vi "Main Page.vi"(8 "error in (no error)":errorcluster, 11 "Node Ptr":T1 format="%.0x") -> (0 "error out":errorcluster)   [LabVIEW 2015, in "Protection and Counter Addon System Explorer.lvlib"]
uses:
  Protection and Counter Addon System Explorer.lvlib
  <vilib>/NI Veristand/Custom Device API/Custom Device Item Ref.ctl
  <vilib>/NI/Hardware Resource Discovery/Types/Filter Type.ctl
  Shared/Types/986x.ctl
  Shared/SubVIs/GUID Lookup.vi
  <vilib>/NI Veristand/Custom Device API/NI VeriStand - Get Item Property.vi
  <vilib>/NI Veristand/Custom Device API/Get Item Property (Boolean).vi
  <vilib>/NI Veristand/Custom Device API/Get Item Property (String).vi
  <vilib>/NI Veristand/Custom Device API/Get Item Property (Dependent File).vi
  <vilib>/NI VeriStand/Custom Device API/Custom Device API.lvlib
  <vilib>/NI/Hardware Resource Discovery/NIVS Hardware Discovery.lvlib
  Shared/Protection and Counter Addon Shared.lvlib
panel:
  in  "FPGA Settings":cluster{"Section Name":string}={"Section Name"="FPGA Settings"}
  in  "RIO Browse":bool
  in  "RIO Device":string
  in  "Enable Bitfile":bool
  in  "Bitfile Path":path
  in  "Use Legacy":bool
  in  "Loop Priority":i32=100 format="%.0p"
  in  "FD Baud rate [Bd]":u64 format="%.0p"
  in  "CAN I/O Mode":u32(ring) items=["CAN 2.0", "CAN FD", "CAN FD+BRS"]
  in  "Database Settings":cluster{"Section Name":string}={"Section Name"="Database Settings"}
  in  "CAN Browse":bool
  in  "Termination":enum16{"Off", "On"}(ring)
  in  "CAN Port":string
  in  "Baud rate [Bd]":u64 format="%.0p"
  out "XNET Cluster":refnum<k21>
  out "XNET Database":refnum<k21>
  in  "SHDocVw.IWebBrowser2":refnum<k7>(container)
  in  "Header":cluster{"Section Name":string}={"Section Name"="CAN Settings"}
  in  "Name":string
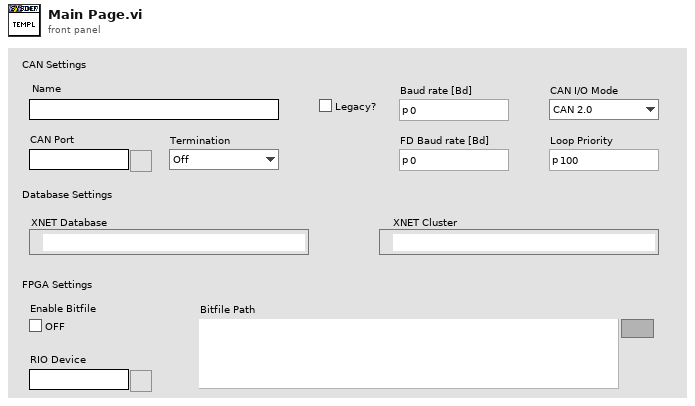
[diagram p1: front panel]
types:
  T1 = typedef "Custom Device API.lvlib/Custom Device Item Ref.ctl" = u64
  T2 = typedef "Protection and Counter Addon Shared.lvlib/986x.ctl" = cluster{"Enable":bool, "RIO Device":string, "Bitfile":path}
  T3 = typedef "Protection and Counter Addon Shared.lvlib/XNET Settings.ctl" = cluster{"Database":refnum<k21>, "Cluster":refnum<k21>, "Port":string, "Baud rate [Bd]":u64, "Termination":u32, "CAN I/O Mode":u32, "FD Baud rate [Bd]":u64, "Priority":i32, "Use Legacy":bool}
  T4 = typedef "Custom Device API.lvlib/Custom Device Item Info.ctl" = cluster{"Name":string, "Is Channel":bool, "GUID":string, "Is Waveform":bool}
  T5 = typedef "NIVS Hardware Discovery.lvlib/Filter Type.ctl" = enum16{"Device Category", "Product Name", "Ethernet", "XNET", "VISA", "FPGA", "EtherCAT Master", "DAQmx", "GPIB", "Serial"}
  T6 = typedef "Custom Device API.lvlib/Custom Device Commands.ctl" = enum16{"Default", "Item renamed", "Shutdown", "Dynamic button pressed"}
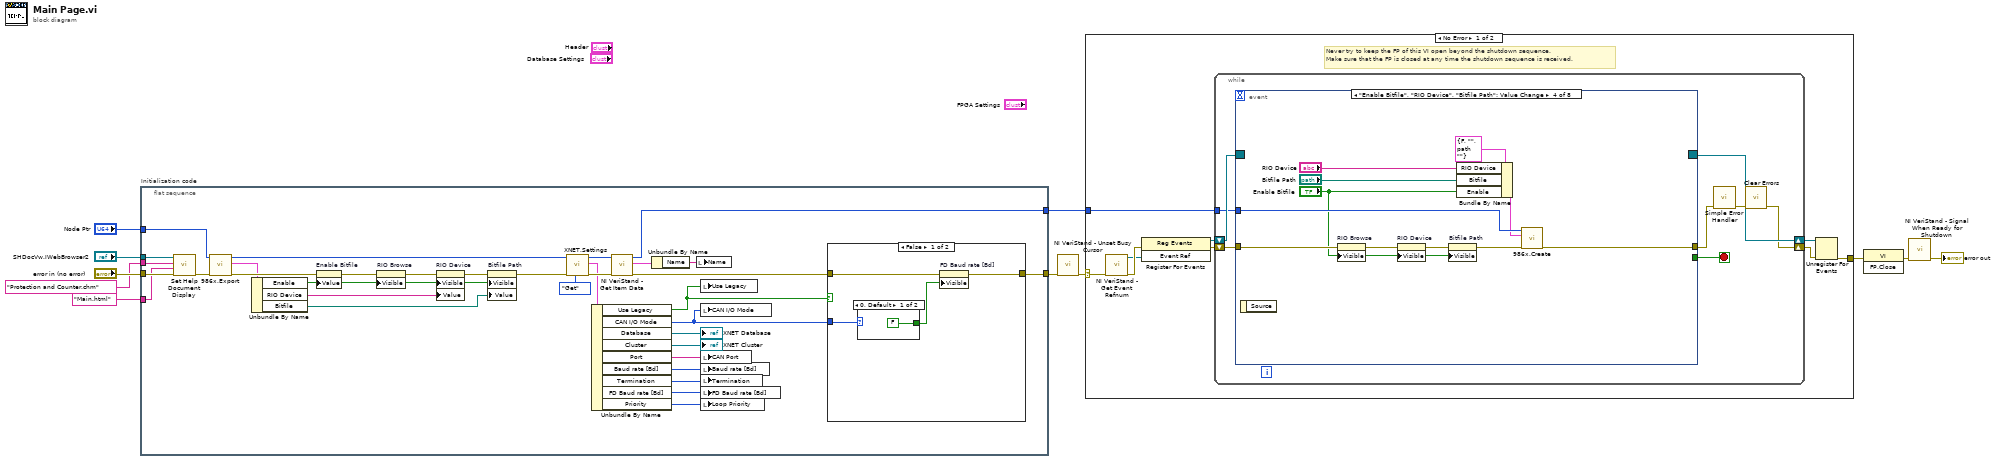
[diagram p0: block diagram]
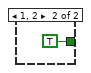
[diagram p2: hidden frame]
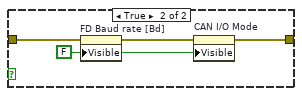
[diagram p3: hidden frame]
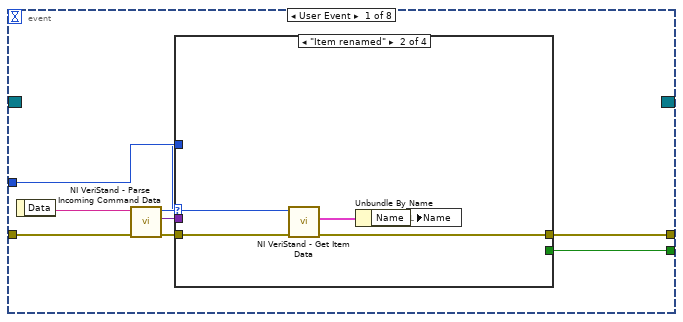
[diagram p4: hidden frame]
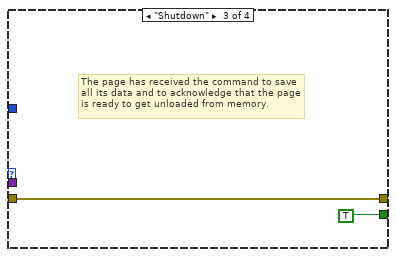
[diagram p6: hidden frame]
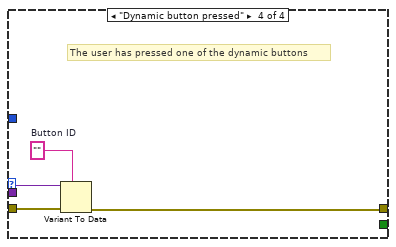
[diagram p7: hidden frame]
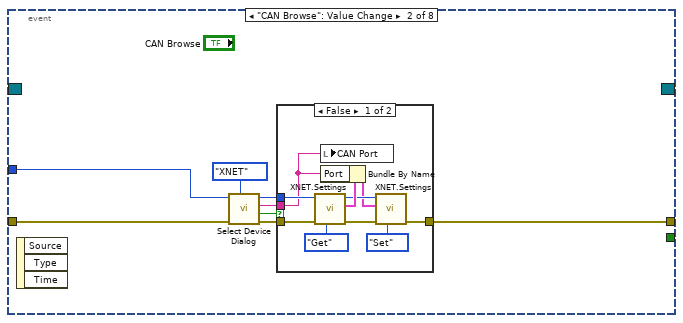
[diagram p8: hidden frame]
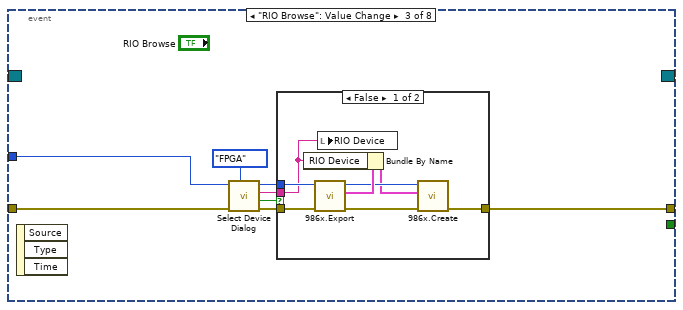
[diagram p10: hidden frame]
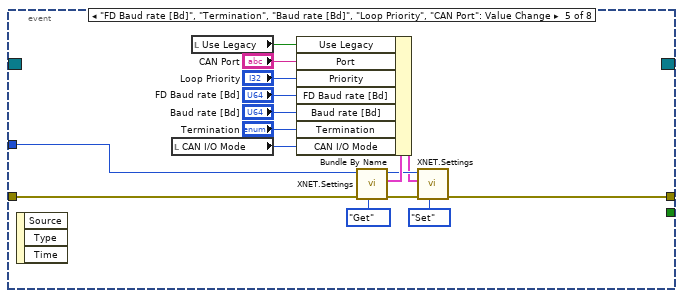
[diagram p12: hidden frame]
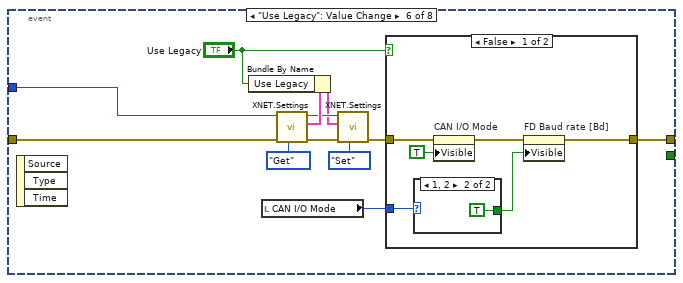
[diagram p13: hidden frame]
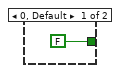
[diagram p14: hidden frame]
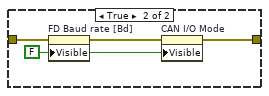
[diagram p15: hidden frame]
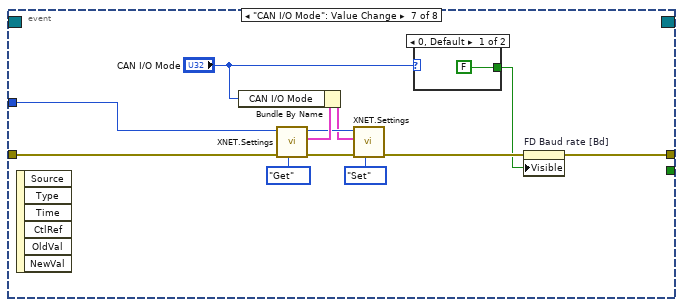
[diagram p16: hidden frame]
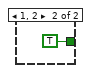
[diagram p17: hidden frame]
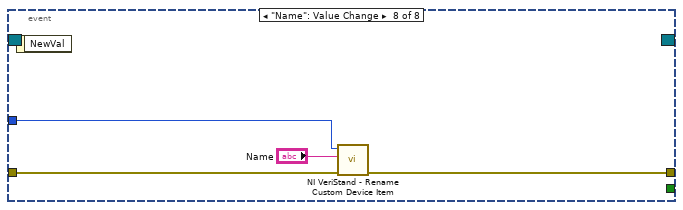
[diagram p18: hidden frame]
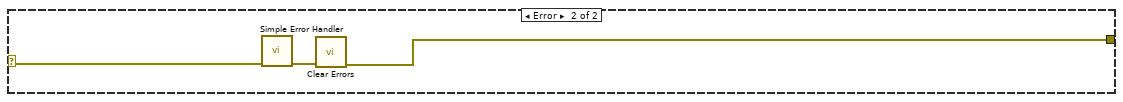
[diagram p19: hidden frame]
diagram:
  n1 = flat-sequence "Initialization code" {
    tunnel: "error in (no error)" -> [w42]
    tunnel: "Node Ptr" -> [w22]
    tunnel: [w25] -> w7
    tunnel: [w45] -> w4
    tunnel: "SHDocVw.IWebBrowser2" -> [w41]
    tunnel: "Protection and Counter.chm" ("Main CHM File") -> [w40]
    tunnel: "Main.html" ("HTML File") -> [w39]
    frame #0 {
      n2 = call "Set Help Document Display.vi"("error in (no error)"=w42, "HTML File"=w39, "Main CHM File"=w40, "SHDocVw.IWebBrowser2"=w41) -> ("error out"=w23:errorcluster)  [unwired: 7 in]
      n3 = call "986x.Export.vi"("error in (no error)"=w23, "Device Item Ref in"=w22) -> ("error out"=w17:errorcluster, "986x Support"=w15:T2, "Item Ref out"=w21:T1)  [unwired: 7 in]
      n4 = Unbundle By Name(w15) -> ("Enable"=w14:bool, "RIO Device"=w13:string, "Bitfile"=w12:path)
      n5 = property on="Enable Bitfile" class="Bool (strict)"(error in=w17, "Value"=w14) -> (error out=w20:errorcluster)  [unwired: 1 in, 1 out]
      n6 = property on="RIO Browse" class="Bool"(error in=w20, "Visible"=w14) -> (error out=w19:errorcluster)  [unwired: 1 in, 1 out]
      n7 = property on="RIO Device" class="Str"(error in=w19, "Visible"=w14, "Value"=w13) -> (error out=w18:errorcluster)  [unwired: 1 in, 1 out]
      n8 = property on="Bitfile Path" class="Path"(error in=w18, "Visible"=w14, "Value"=w12) -> (error out=w16:errorcluster)  [unwired: 1 in, 1 out]
      n9 = call "XNET.Settings.vi"("Action"=enum8{"Get", "Set"}."Get", "error in (no error)"=w16, "Parent Ref in"=w21) -> ("error out"=w38:errorcluster, "XNET Settings"=w35:T3, "Item Ref out"=w37:T1)  [unwired: 6 in]
      n10 = Unbundle By Name(w35) -> ("Use Legacy"=w27:bool, "CAN I/O Mode"=w24:u32, "Database"=→"XNET Database":refnum<k21>, "Cluster"=→"XNET Cluster":refnum<k21>, "Port"=w32:string, "Baud rate [Bd]"=w31:u64, "Termination"=w30:u32, "FD Baud rate [Bd]"=w29:u64, "Priority"=w28:i32)
      n11 = call <vilib>:"NI VeriStand - Get Item Data.vi"("error in (no error)"=w38, "Item Ref in"=w37) -> ("error out"=w26:errorcluster, "Item Info"=w44:T4, "Item Ref out"=w45:T1)  [unwired: 7 out]
      n12 = Unbundle By Name(w44) -> ("Name"=w43:string)
      n13 = local write "Name"(w43) -> ()
      n14 = local write "Use Legacy"(w27) -> ()
      n15 = local write "CAN I/O Mode"(w24) -> ()
      n16 = local write "CAN Port"(w32) -> ()
      n17 = local write "Baud rate [Bd]"(w31) -> ()
      n18 = local write "Termination"(w30) -> ()
      n19 = local write "FD Baud rate [Bd]"(w29) -> ()
      n20 = local write "Loop Priority"(w28) -> ()
      n21 = case shown="False" w27 {
        tunnel: w26 -> [w48 w54]
        tunnel: [w47 w53] -> w25
        tunnel: w24 -> [w49 _]
        frame False {
          n22 = case shown="0, Default" w49 {
            tunnel: [FALSE TRUE] -> w46
            frame 0, Default {
            }
            frame 1, 2 {
            }
          }
          n23 = property on="FD Baud rate [Bd]" class="DigNum (strict)"(error in=w48, "Visible"=w46) -> (error out=w47:errorcluster)  [unwired: 1 in, 1 out]
        }
        frame True {
          w52 = FALSE ("Visible")
          n24 = property on="FD Baud rate [Bd]" class="DigNum (strict)"(error in=w54, "Visible"=w52) -> (error out=w55:errorcluster)  [unwired: 1 in, 1 out]
          n25 = property on="CAN I/O Mode" class="Ring (strict)"(error in=w55, "Visible"=w52) -> (error out=w53:errorcluster)  [unwired: 1 in, 1 out]
        }
      }
    }
  }
  n26 = call <vilib>:"NI VeriStand - Unset Busy Cursor.vi"("error in (no error)"=w7) -> ("error out"=w6:errorcluster)  [unwired: 10 out]
  n27 = case shown="No Error" w6 {
    selector: w6 -> [w56 w200]
    tunnel: [w61 w198] -> w11
    tunnel: w4 -> [w57 _]
    frame No Error {
      # "Never try to keep the FP of this VI open beyond the shutdown sequence.\nMake sure that the FP is closed at any time the shutdown sequence is received."
      n28 = call <vilib>:"NI VeriStand - Get Event Refnum.vi"("error in (no error)"=w56) -> ("error out"=w64:errorcluster, "Event Ref"=w60:refnum<user-event>)  [unwired: 9 out]
      n29 = register-events(error in=w64, w60) -> (reference out=w58:refnum<event-registration>, error out=w59:errorcluster)  [unwired: 1 in]
      n30 = while {
        tunnel: w57 -> [w68]
        shift-right: [w65] -> w62
        shift-left: w59 -> [w71]
        shift-right: [w72] -> w63
        shift-left: w58 -> [w70]
        stop <- w69 stop-if-true
        n31 = event shown="[3] \"Enable Bitfile\", \"RIO Device\", \"Bitfile Path\": Value Change" {
          selector: w70 -> [_ _ _ _ _ _ _ _]
          dyn-events: [_ _ _ _ _ _ _ _] -> w72
          timeout: _ -> [_ _ _ _ _ _ _ _]
          tunnel: w71 -> [w80 w95 w114 w136 w149 w161 w185 w197]
          tunnel: [w76 _ _ _ _ _ _ _] -> w69
          tunnel: [w75 w93 w112 w139 w148 w157 w182 w196] -> w67
          tunnel: w68 -> [w74 w94 w113 w134 w147 w160 w184 w195]
          event User Event {
            n32 = event-data() -> ("Data"=w79:string)  [unwired: 1 out]
            n33 = call <vilib>:"NI VeriStand - Parse Incoming Command Data.vi"("error in (no error)"=w80, "Incoming data"=w79) -> ("error out"=w78:errorcluster, "Outgoing data"=w73:variant, "Action"=w77:T6)  [unwired: 7 out]
            n34 = case shown="\"Item renamed\"" w77 {
              tunnel: w78 -> [w81 w86 w87 w92]
              tunnel: [_ _ TRUE _] -> w76
              tunnel: [w81 w83 w87 w89] -> w75
              tunnel: w74 -> [_ w85 _ _]
              tunnel: w73 -> [_ _ _ w91]
              frame "Default", Default {
              }
              frame "Item renamed" {
                n35 = call <vilib>:"NI VeriStand - Get Item Data.vi"("error in (no error)"=w86, "Item Ref in"=w85) -> ("error out"=w83:errorcluster, "Item Info"=w84:T4)  [unwired: 8 out]
                n36 = Unbundle By Name(w84) -> ("Name"=w82:string)
                n37 = local write "Name"(w82) -> ()
              }
              frame "Shutdown" {
                # "The page has received the command to save all its data and to acknowledge that the page is ready to get unloaded from memory."
              }
              frame "Dynamic button pressed" {
                w90 = ""  # Button ID
                # "The user has pressed one of the dynamic buttons"
                n38 = Variant To Data(error in=w92, type=w90, Variant=w91) -> (error out=w89:errorcluster)  [unwired: 1 out]
              }
            }
          }
          event "CAN Browse": Value Change {
            n39 = event-data() -> ()  [unwired: 4 out]
            n40 = call <vilib>:"Select Device Dialog.vi"("Filter Type"=Filter_Type."XNET", "error in (no error)"=w95, "Item Ref in"=w94) -> ("error out"=w99:errorcluster, "Cancelled?"=w98:bool, "Selected Alias"=w97:string, "Item Ref out"=w100:T1)  [unwired: 5 in]
            n41 = case shown="False" w98 {
              tunnel: w100 -> [w108 _]
              tunnel: [w105 w111] -> w93
              tunnel: w99 -> [w102 w111]
              tunnel: w97 -> [w101 _]
              frame False {
                n42 = call "XNET.Settings.vi"("Action"=enum8{"Get", "Set"}."Get", "error in (no error)"=w102, "Parent Ref in"=w108) -> ("error out"=w103:errorcluster, "XNET Settings"=w109:T3, "Item Ref out"=w106:T1)  [unwired: 6 in]
                n43 = local write "CAN Port"(w101) -> ()
                n44 = Bundle By Name(cluster=w109, "Port"=w101) -> (w104:T3)
                n45 = call "XNET.Settings.vi"("Action"=enum8{"Get", "Set"}."Set", "error in (no error)"=w103, "XNET Settings"=w104, "Parent Ref in"=w106) -> ("error out"=w105:errorcluster)  [unwired: 5 in, 2 out]
              }
              frame True {
              }
            }
          }
          event "RIO Browse": Value Change {
            n46 = event-data() -> ()  [unwired: 4 out]
            n47 = call <vilib>:"Select Device Dialog.vi"("Filter Type"=Filter_Type."FPGA", "error in (no error)"=w114, "Item Ref in"=w113) -> ("error out"=w118:errorcluster, "Cancelled?"=w117:bool, "Selected Alias"=w116:string, "Item Ref out"=w119:T1)  [unwired: 5 in]
            n48 = case shown="False" w117 {
              tunnel: w119 -> [w126 _]
              tunnel: [w121 w128] -> w112
              tunnel: w118 -> [w125 w128]
              tunnel: w116 -> [w124 _]
              frame False {
                n49 = call "986x.Export.vi"("error in (no error)"=w125, "Device Item Ref in"=w126) -> ("error out"=w123:errorcluster, "986x Support"=w127:T2, "Item Ref out"=w122:T1)  [unwired: 7 in]
                n50 = Bundle By Name(cluster=w127, "RIO Device"=w124) -> (w120:T2)
                n51 = local write "RIO Device"(w124) -> ()
                n52 = call "986x.Create.vi"("error in (no error)"=w123, "986x Support"=w120, "Device Item Ref in"=w122) -> ("error out"=w121:errorcluster)  [unwired: 7 in, 1 out]
              }
              frame True {
              }
            }
          }
          event "Enable Bitfile", "RIO Device", "Bitfile Path": Value Change {
            n53 = event-data() -> ()  [unwired: 2 out]
            n54 = property on="RIO Browse" class="Bool"(error in=w136, "Visible"="Enable Bitfile") -> (error out=w137:errorcluster)  [unwired: 1 in, 1 out]
            n55 = property on="RIO Device" class="Str"(error in=w137, "Visible"="Enable Bitfile") -> (error out=w138:errorcluster)  [unwired: 1 in, 1 out]
            n56 = property on="Bitfile Path" class="Path"(error in=w138, "Visible"="Enable Bitfile") -> (error out=w135:errorcluster)  [unwired: 1 in, 1 out]
            n57 = Bundle By Name(cluster=T2 {"Enable"=FALSE, "RIO Device"="", "Bitfile"=path ""} ("986x Support"), "RIO Device"="RIO Device", "Bitfile"="Bitfile Path", "Enable"="Enable Bitfile") -> (w132:T2)
            n58 = call "986x.Create.vi"("error in (no error)"=w135, "986x Support"=w132, "Device Item Ref in"=w134) -> ("error out"=w139:errorcluster)  [unwired: 7 in, 1 out]
          }
          event "FD Baud rate [Bd]", "Termination", "Baud rate [Bd]", "Loop Priority", "CAN Port": Value Change {
            n59 = event-data() -> ()  [unwired: 4 out]
            n60 = local read "CAN I/O Mode"() -> (w140:u32)
            n61 = local read "Use Legacy"() -> (w141:bool)
            n62 = call "XNET.Settings.vi"("Action"=enum8{"Get", "Set"}."Get", "error in (no error)"=w149, "Parent Ref in"=w147) -> ("error out"=w150:errorcluster, "XNET Settings"=w154:T3, "Item Ref out"=w152:T1)  [unwired: 6 in]
            n63 = Bundle By Name(cluster=w154, "Use Legacy"=w141, "Port"="CAN Port", "Priority"="Loop Priority", "FD Baud rate [Bd]"="FD Baud rate [Bd]", "Baud rate [Bd]"="Baud rate [Bd]", "Termination"="Termination", "CAN I/O Mode"=w140) -> (w151:T3)
            n64 = call "XNET.Settings.vi"("Action"=enum8{"Get", "Set"}."Set", "error in (no error)"=w150, "XNET Settings"=w151, "Parent Ref in"=w152) -> ("error out"=w148:errorcluster)  [unwired: 5 in, 2 out]
          }
          event "Use Legacy": Value Change {
            n65 = event-data() -> ()  [unwired: 4 out]
            n66 = local read "CAN I/O Mode"() -> (w156:u32)
            n67 = call "XNET.Settings.vi"("Action"=enum8{"Get", "Set"}."Get", "error in (no error)"=w161, "Parent Ref in"=w160) -> ("error out"=w162:errorcluster, "XNET Settings"=w166:T3, "Item Ref out"=w164:T1)  [unwired: 6 in]
            n68 = Bundle By Name(cluster=w166, "Use Legacy"="Use Legacy") -> (w163:T3)
            n69 = call "XNET.Settings.vi"("Action"=enum8{"Get", "Set"}."Set", "error in (no error)"=w162, "XNET Settings"=w163, "Parent Ref in"=w164) -> ("error out"=w158:errorcluster)  [unwired: 5 in, 2 out]
            n70 = case shown="False" "Use Legacy" {
              tunnel: w158 -> [w170 w178]
              tunnel: [w173 w177] -> w157
              tunnel: w156 -> [w171 _]
              frame False {
                n71 = case shown="1, 2" w171 {
                  tunnel: [FALSE TRUE] -> w172
                  frame 0, Default {
                  }
                  frame 1, 2 {
                  }
                }
                n72 = property on="CAN I/O Mode" class="Ring (strict)"(error in=w170, "Visible"=TRUE) -> (error out=w169:errorcluster)  [unwired: 1 in, 1 out]
                n73 = property on="FD Baud rate [Bd]" class="DigNum (strict)"(error in=w169, "Visible"=w172) -> (error out=w173:errorcluster)  [unwired: 1 in, 1 out]
              }
              frame True {
                w176 = FALSE ("Visible")
                n74 = property on="FD Baud rate [Bd]" class="DigNum (strict)"(error in=w178, "Visible"=w176) -> (error out=w179:errorcluster)  [unwired: 1 in, 1 out]
                n75 = property on="CAN I/O Mode" class="Ring (strict)"(error in=w179, "Visible"=w176) -> (error out=w177:errorcluster)  [unwired: 1 in, 1 out]
              }
            }
          }
          event "CAN I/O Mode": Value Change {
            n76 = event-data() -> ()  [unwired: 7 out]
            n77 = call "XNET.Settings.vi"("Action"=enum8{"Get", "Set"}."Get", "error in (no error)"=w185, "Parent Ref in"=w184) -> ("error out"=w186:errorcluster, "XNET Settings"=w190:T3, "Item Ref out"=w188:T1)  [unwired: 6 in]
            n78 = Bundle By Name(cluster=w190, "CAN I/O Mode"="CAN I/O Mode") -> (w187:T3)
            n79 = call "XNET.Settings.vi"("Action"=enum8{"Get", "Set"}."Set", "error in (no error)"=w186, "XNET Settings"=w187, "Parent Ref in"=w188) -> ("error out"=w183:errorcluster)  [unwired: 5 in, 2 out]
            n80 = case shown="0, Default" "CAN I/O Mode" {
              tunnel: [FALSE TRUE] -> w181
              frame 0, Default {
              }
              frame 1, 2 {
              }
            }
            n81 = property on="FD Baud rate [Bd]" class="DigNum (strict)"(error in=w183, "Visible"=w181) -> (error out=w182:errorcluster)  [unwired: 1 in, 1 out]
          }
          event "Name": Value Change {
            n82 = event-data() -> ()  [unwired: 2 out]
            n83 = call <vilib>:"NI VeriStand - Rename Custom Device Item.vi"("error in (no error)"=w197, "New Name"="Name", "Item Ref in"=w195) -> ("error out"=w196:errorcluster)  [unwired: 1 in, 7 out]
          }
        }
        n84 = call <vilib>:"Simple Error Handler.vi"("error in (no error)"=w67) -> ("error out"=w66:errorcluster)  [unwired: 1 in, 7 out]
        n85 = call <vilib>:"Clear Errors.vi"("error in (no error)"=w66) -> ("error out"=w65:errorcluster)  [unwired: 1 in, 5 out]
      }
      n86 = Unregister For Events(event registration refnum=w63, error in=w62) -> (error out=w61:errorcluster)
    }
    frame Error {
      n87 = call <vilib>:"Simple Error Handler.vi"("error in (no error)"=w200) -> ("error out"=w199:errorcluster)  [unwired: 1 in, 7 out]
      n88 = call <vilib>:"Clear Errors.vi"("error in (no error)"=w199) -> ("error out"=w198:errorcluster)  [unwired: 1 in, 5 out]
    }
  }
  n89 = invoke class="VI" method="FP.Close"(error in=w11) -> (error out=w10:errorcluster)  [unwired: 2 in, 2 out]
  n90 = call <vilib>:"NI VeriStand - Signal When Ready for Shutdown.vi"("error in (no error)"=w10) -> ("error out"=→"error out":errorcluster)  [unwired: 10 out]
